vi "get channels.vi"(11 "E2E configuration in":refnum<class "E2E Tag Exchange configuration.lvclass">) -> (2 "channels":refnum<class "TBM channel.lvclass">[](array[class]), 3 "E2E configuration out":refnum<class "E2E Tag Exchange configuration.lvclass">)   [LabVIEW 2015, in "E2E Tag Exchange configuration.lvclass"]
doc: "Returns an array of all Channels currently added to this configuration object."
uses:
  E2E Tag Exchange configuration.lvclass
  <vilib>/NI/Tag Bus Module Framework/channel/TBM channel.lvclass
  E2E Tag Exchange configuration.lvclass/E2E Tag Exchange configuration.ctl
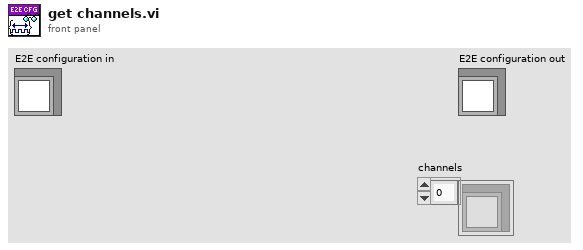
[diagram p1: front panel]
types:
  T1 = typedef "E2E Tag Exchange configuration.lvclass/Runtime Implementation.ctl" = enum16{"RT FIFO", "UDP"}
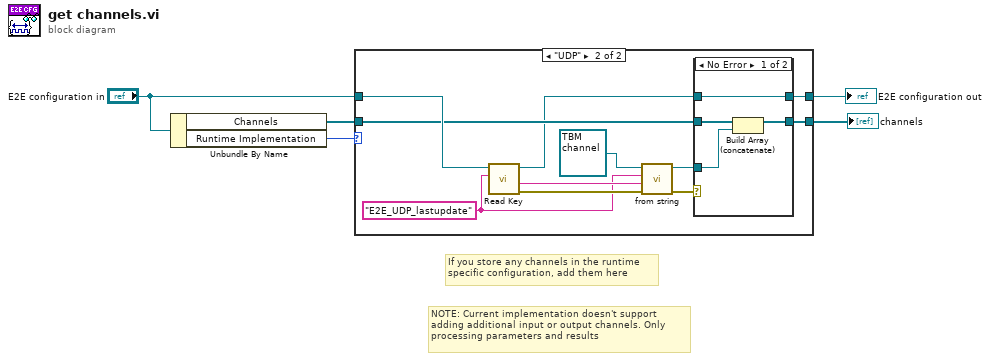
[diagram p0: block diagram]
diagram:
  # "NOTE: Current implementation doesn't support\nadding additional input or output channels. Only\nprocessing parameters and results"
  # "If you store any channels in the runtime\nspecific configuration, add them here"
  n1 = Unbundle By Name("E2E configuration in") -> ("Channels"=w5:refnum<class "TBM channel.lvclass">[], "Runtime Implementation"=w4:T1)
  n2 = case shown="\"UDP\"" w4 {
    tunnel: w5 -> [w7 w12]
    tunnel: [w7 w10] -> w3
    tunnel: "E2E configuration in" -> [w6 w14]
    tunnel: [w6 w8] -> w1
    frame "RT FIFO" {
    }
    frame "UDP" {
      w16 = "E2E_UDP_lastupdate" ("Key")
      n3 = call "Read Key.vi"("Key"=w16, "E2E configuration in"=w14) -> ("error out"=w17:errorcluster, "Value"=w18:string, "E2E configuration out"=w9:refnum<class "E2E Tag Exchange configuration.lvclass">)  [unwired: 7 in]
      n4 = call-dynamic "from string.vi"("error in"=w17, "channel data"=w18, "identifier"=w16, "channel in"=refnum<class "TBM channel.lvclass"> refnum) -> ("error out"=w13:errorcluster, "channel out"=w11:refnum<class "TBM channel.lvclass">)  [unwired: 6 in]
      n5 = case shown="No Error" w13 {
        tunnel: w12 -> [w22 w24]
        tunnel: w11 -> [w21 _]
        tunnel: [w20 w24] -> w10
        tunnel: w9 -> [w19 w23]
        tunnel: [w19 w23] -> w8
        frame No Error {
          n6 = Build Array (concatenate)(w22, w21) -> (w20:refnum<class "TBM channel.lvclass">[])
        }
        frame Error {
        }
      }
    }
  }
  "E2E configuration out" <- w1
  "channels" <- w3
